vi "add and map fixed channel mapping.vi"(5 "set module as owner":bool, 7 "module instance":string, 8 "error in":errorcluster, 10 "fixed channel":refnum<class "TBM channel.lvclass">, 11 "engine configuration in":refnum<class "engine configuration.lvclass">) -> (0 "error out":errorcluster, 3 "engine configuration out":refnum<class "engine configuration.lvclass">)   [LabVIEW 2014, in "engine configuration.lvclass"]
doc: "This function will automatically generate a new tag with the same name as the input channel and that channel to the newly created tag. If the channel is already mapped, or if a tag with that name already exists, the function will return without error."
uses:
  engine configuration.lvclass
  <vilib>/NI/Tag Bus Module Framework/channel/TBM channel.lvclass
  <vilib>/NI/Tag Bus/tag/tag descriptor.lvclass/tag descriptor.ctl
  <vilib>/NI/Tag Bus/tag/read tag name.vi
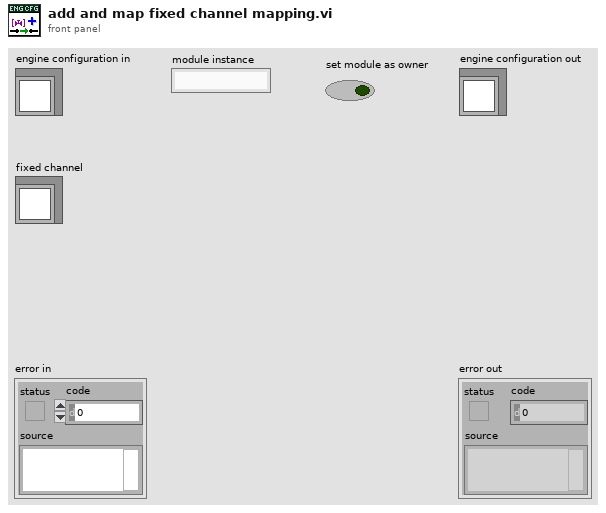
[diagram p1: front panel]
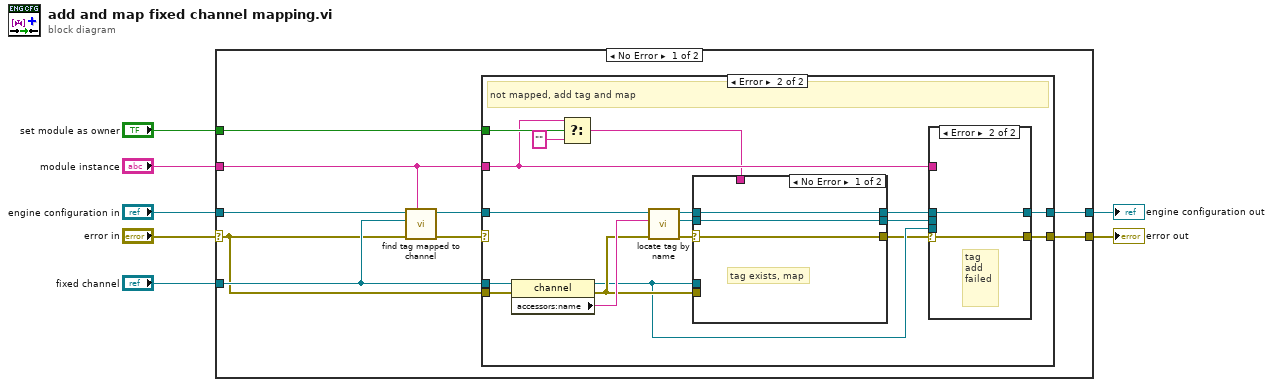
[diagram p0: block diagram]
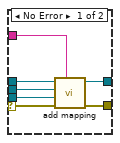
[diagram p3: hidden frame]
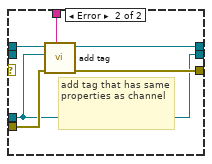
[diagram p4: hidden frame]
diagram:
  n1 = case shown="No Error" "error in" {
    selector: "error in" -> [w9 w56]
    tunnel: [w11 w56] -> w6
    tunnel: [w12 w55] -> w4
    tunnel: "engine configuration in" -> [w16 w55]
    tunnel: "fixed channel" -> [w10 _]
    tunnel: "module instance" -> [w15 _]
    tunnel: "set module as owner" -> [w8 _]
    frame No Error {
      n2 = call "find tag mapped to channel.vi"("owner"=w15, "error in"=w9, "channel"=w10, "engine configuration in"=w16) -> ("error out"=w14:errorcluster, "engine configuration out"=w13:refnum<class "engine configuration.lvclass">)  [unwired: 5 in, 1 out]
      n3 = case shown="Error" w14 {
        selector: w14 -> [w17 _]
        tunnel: w15 -> [_ w21]
        tunnel: w10 -> [_ w36]
        tunnel: w9 -> [_ w35]
        tunnel: w13 -> [w18 w33]
        tunnel: [w18 w27] -> w12
        tunnel: [w17 w26] -> w11
        tunnel: w8 -> [_ w22]
        frame No Error {
          # "Already mapped, do nothing"
        }
        frame Error {
          # "not mapped, add tag and map"
          n4 = property class="channel"(reference=w36, error in=w35) -> (reference out=w24:refnum<class "TBM channel.lvclass">, error out=w31:errorcluster, "accessors:name"=w34:string)
          n5 = Select(t=w21, s=w22, f="") -> (s? t:f=w19:string)
          n6 = call "locate tag by name.vi"("error in"=w31, "tag name"=w34, "engine configuration in"=w33) -> ("error out"=w32:errorcluster, "tag descriptor"=w30:refnum<class "tag descriptor.lvclass">, "engine configuration out"=w29:refnum<class "engine configuration.lvclass">)  [unwired: 6 in]
          n7 = case shown="No Error" w32 {
            selector: w32 -> [w46 _]
            tunnel: w31 -> [_ w52]
            tunnel: w19 -> [_ w53]
            tunnel: [w48 w49] -> w25
            tunnel: w30 -> [w48 _]
            tunnel: w29 -> [w47 w54]
            tunnel: [w47 w51] -> w28
            tunnel: [w46 w50] -> w23
            tunnel: w24 -> [_ w49]
            frame No Error {
              # "tag exists, map"
            }
            frame Error {
              # "add tag that has same properties as channel"
              n8 = call-dynamic "add tag.vi"("owner ID"=w53, "error in"=w52, "tag descriptor"=w49, "engine configuration in"=w54) -> ("error out"=w50:errorcluster, "engine configuration out"=w51:refnum<class "engine configuration.lvclass">)  [unwired: 6 in]
            }
          }
          n9 = case shown="Error" w23 {
            selector: w23 -> [w37 w44]
            tunnel: w28 -> [w43 w45]
            tunnel: [w42 w45] -> w27
            tunnel: [w41 w44] -> w26
            tunnel: w25 -> [w40 _]
            tunnel: w21 -> [w39 _]
            tunnel: w24 -> [w38 _]
            frame No Error {
              n10 = call-dynamic "add mapping.vi"("owner ID"=w39, "error in"=w37, "channel"=w38, "tag descriptor"=w40, "engine configuration"=w43) -> ("error out"=w41:errorcluster, "engine configuration out"=w42:refnum<class "engine configuration.lvclass">)  [unwired: 5 in]
            }
            frame Error {
              # "tag add failed"
            }
          }
        }
      }
    }
    frame Error {
    }
  }
  "error out" <- w6
  "engine configuration out" <- w4
